vi "UI - Initiate IO Var Crio2.vi"(11 "Controller Address":string) -> (3 "IO References":T1)   [LabVIEW 2025]
uses:
  controls/IO References.ctl
panel:
  out "Array":string[](array[string])
  out "Array 2":errorcluster[](array[cluster])
  out "error out":errorcluster
  in  "error in (no error)":errorcluster
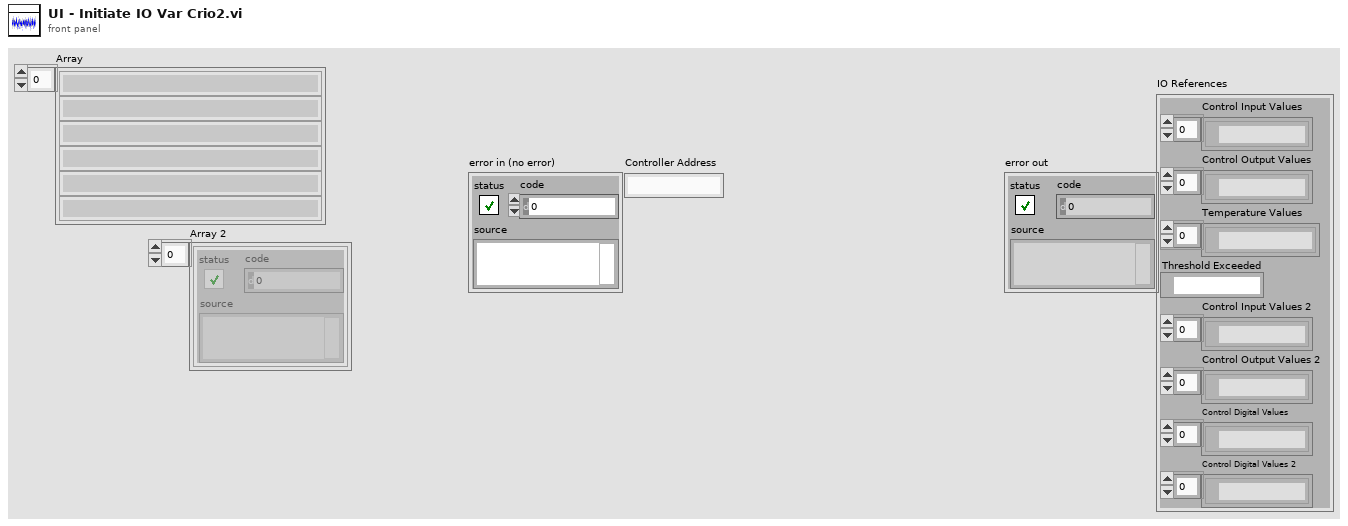
[diagram p1: front panel]
types:
  T1 = typedef "IO References.ctl" = cluster{"Control Input Values":refnum<k21>[], "Control Output Values":refnum<k21>[], "Temperature Values":refnum<k21>[], "Threshold Exceeded":refnum<k21>, "Control Input Values 2":refnum<k21>[], "Control Output Values 2":refnum<k21>[], "Control Digital Values":refnum<k21>[], "Control Digital Values 2":refnum<k21>[]}
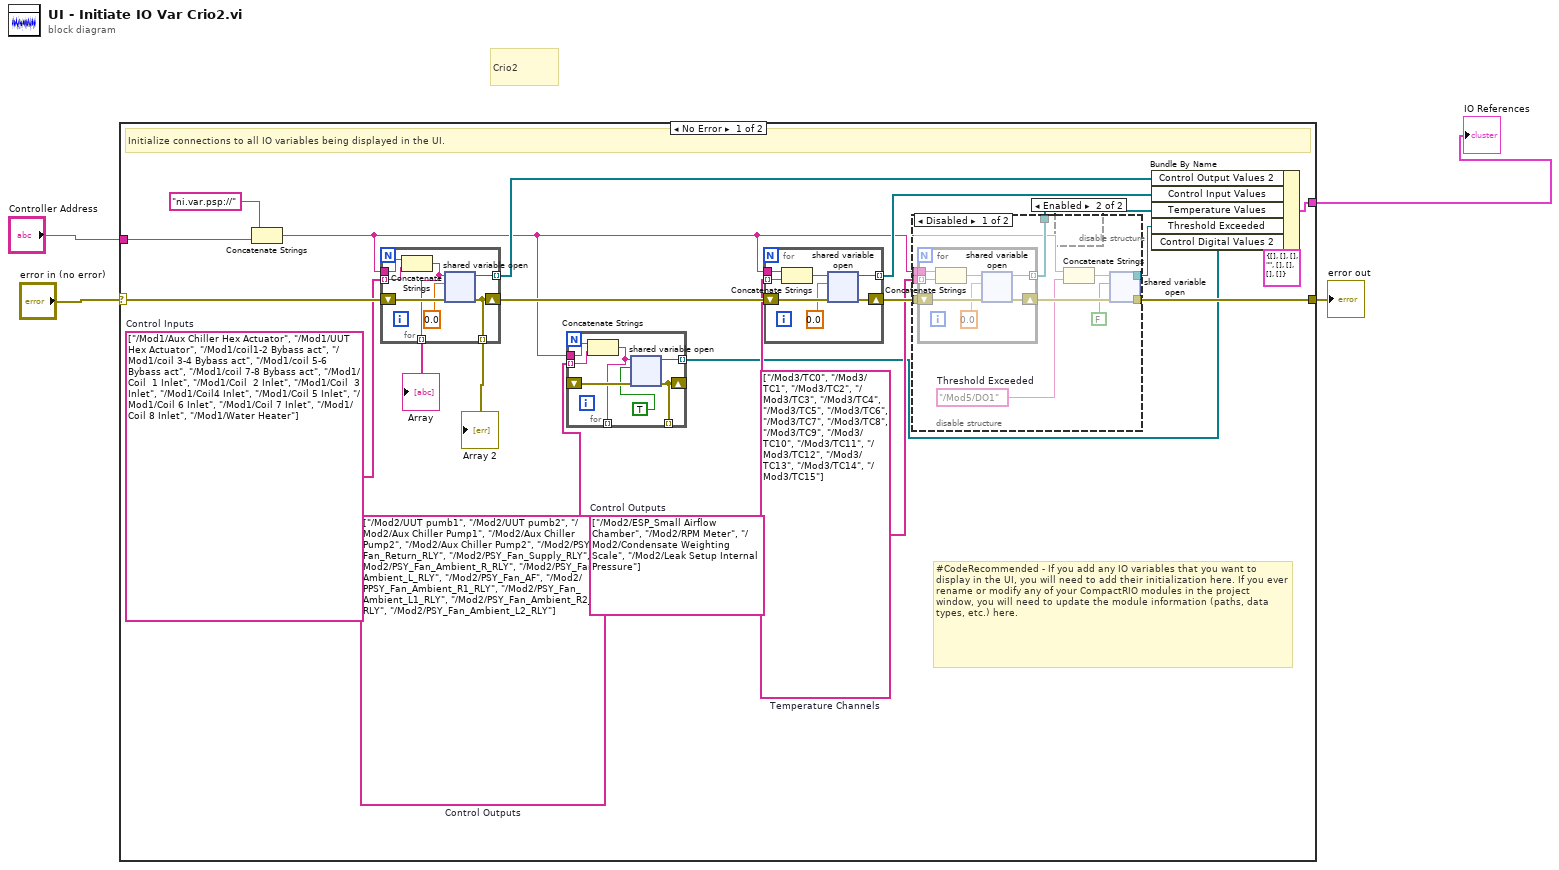
[diagram p0: block diagram]
diagram:
  # "Crio2"
  n1 = case shown="No Error" "error in (no error)" {
    selector: "error in (no error)" -> [w21 w64]
    tunnel: "Controller Address" -> [w23 _]
    tunnel: [w10 w64] -> w2
    tunnel: [w18 _] -> w1
    frame No Error {
      w5 = string[] ["/Mod2/UUT pumb1", "/Mod2/UUT pumb2", "/Mod2/Aux Chiller Pump1", "/Mod2/Aux Chiller Pump2", "/Mod2/Aux Chiller Pump2", "/Mod2/PSY_Fan_Return_RLY", "/Mod2/PSY_Fan_Supply_RLY", "/Mod2/PSY_Fan_Ambient_R_RLY", "/Mod2/PSY_Fan_Ambient_L_RLY", "/Mod2/PSY_Fan_AF", "/Mod2/PPSY_Fan_Ambient_R1_RLY", "/Mod2/PSY_Fan_Ambient_L1_RLY", "/Mod2/PSY_Fan_Ambient_R2_RLY", "/Mod2/PSY_Fan_Ambient_L2_RLY"]  # Control Outputs
      w13 = string[] ["/Mod3/TC0", "/Mod3/TC1", "/Mod3/TC2", "/Mod3/TC3", "/Mod3/TC4", "/Mod3/TC5", "/Mod3/TC6", "/Mod3/TC7", "/Mod3/TC8", "/Mod3/TC9", "/Mod3/TC10", "/Mod3/TC11", "/Mod3/TC12", "/Mod3/TC13", "/Mod3/TC14", "/Mod3/TC15"]  # Temperature Channels
      w16 = string[] ["/Mod2/ESP_Small Airflow Chamber", "/Mod2/RPM Meter", "/Mod2/Condensate Weighting Scale", "/Mod2/Leak Setup Internal Pressure"]  # Control Outputs
      w20 = string[] ["/Mod1/Aux Chiller Hex Actuator", "/Mod1/UUT Hex Actuator", "/Mod1/coil1-2 Bybass act", "/Mod1/coil 3-4 Bybass act", "/Mod1/coil 5-6 Bybass act", "/Mod1/coil 7-8 Bybass act", "/Mod1/Coil  1 Inlet", "/Mod1/Coil  2 Inlet", "/Mod1/Coil  3 Inlet", "/Mod1/Coil4 Inlet", "/Mod1/Coil 5 Inlet", "/Mod1/Coil 6 Inlet", "/Mod1/Coil 7 Inlet", "/Mod1/Coil 8 Inlet", "/Mod1/Water Heater"]  # Control Inputs
      # "#CodeRecommended - If you add any IO variables that you want to display in the UI, you will need to add their initialization here. If you ever rename or modify any of your CompactRIO modules in the project window, you will need to update the module information (paths, data types, etc.) here."
      # "Initialize connections to all IO variables being displayed in the UI."
      n2 = Concatenate Strings("ni.var.psp://", w23) -> (w7:string)
      n3 = for {
        shift-right: [w57] -> w17
        shift-left: w21 -> [w63]
        tunnel: w7 -> [w61]
        tunnel: w20 -> [w59] mode=indexing
        tunnel: [w60] -> w19 mode=indexing
        tunnel: [w58] -> w9 mode=indexing
        tunnel: [w57] -> w8 mode=indexing
        n4 = Concatenate Strings(w61, w59) -> (w58:string)
        n5 = shared-variable-open(w58, w63, 0.0) -> (w60:refnum<k21>, w57:errorcluster)  [unwired: 1 in]
      }
      "Array" <- w9
      "Array 2" <- w8
      n6 = for {
        shift-right: [w26] -> _
        shift-left: _ -> [w31]
        tunnel: w7 -> [w30]
        tunnel: w5 -> [w28] mode=indexing
        tunnel: [w29] -> w6 mode=indexing
        tunnel: [w27] -> _ mode=indexing
        tunnel: [w26] -> _ mode=indexing
        n7 = Concatenate Strings(w30, w28) -> (w27:string)
        n8 = shared-variable-open(w27, w31, TRUE) -> (w29:refnum<k21>, w26:errorcluster)  [unwired: 1 in]
      }
      n9 = for {
        shift-right: [w55] -> w14
        shift-left: w17 -> [w56]
        tunnel: w7 -> [w52]
        tunnel: w16 -> [w51] mode=indexing
        tunnel: [w50] -> w15 mode=indexing
        n10 = Concatenate Strings(w52, w51) -> (w54:string)
        n11 = shared-variable-open(w54, w56, 0.0) -> (w50:refnum<k21>, w55:errorcluster)  [unwired: 1 in]
      }
      n12 = disable-structure shown="Disabled" {
        disable-tunnel: w14 -> [w41 w49]
        disable-tunnel: w13 -> [w40 _]
        disable-tunnel: [w39 _] -> w12
        disable-tunnel: w7 -> [w38 _]
        disable-tunnel: [w33 _] -> w11
        disable-tunnel: [w32 w49] -> w10
        frame Disabled {
          w36 = "/Mod5/DO1"  # Threshold Exceeded
          n13 = for {
            shift-right: [w47] -> w37
            shift-left: w41 -> [w48]
            tunnel: w38 -> [w44]
            tunnel: w40 -> [w43] mode=indexing
            tunnel: [w42] -> w39 mode=indexing
            n14 = Concatenate Strings(w44, w43) -> (w46:string)
            n15 = shared-variable-open(w46, w48, 0.0) -> (w42:refnum<k21>, w47:errorcluster)  [unwired: 1 in]
          }
          n16 = Concatenate Strings(w38, w36) -> (w35:string)
          n17 = shared-variable-open(w35, w37, FALSE) -> (w33:refnum<k21>, w32:errorcluster)  [unwired: 1 in]
        }
        frame Enabled {
        }
      }
      n18 = disable-structure shown="Enabled" {
        frame Disabled {
        }
        frame Enabled {
        }
      }
      n19 = Bundle By Name(cluster=T1 {"Control Input Values"=[], "Control Output Values"=[], "Temperature Values"=[], "Threshold Exceeded"="", "Control Input Values 2"=[], "Control Output Values 2"=[], "Control Digital Values"=[], "Control Digital Values 2"=[]} ("IO References"), "Control Output Values 2"=w19, "Control Input Values"=w15, "Temperature Values"=w12, "Threshold Exceeded"=w11, "Control Digital Values 2"=w6) -> (w18:T1)
    }
    frame Error {
      # "Error"
    }
  }
  "error out" <- w2
  "IO References" <- w1
